vi "Lab1_task4.vi"() -> ()   [LabVIEW 2022 SP3]
uses:
  <vilib>/Utility/file.llb/Write Delimited Spreadsheet (DBL).vi
panel:
  in  "file path (dialog if empty)":path
  out "Waveform Graph":dbl[](graph)
  in  "Sampling Period (ms)":u32
  in  "Number of Samples":i32
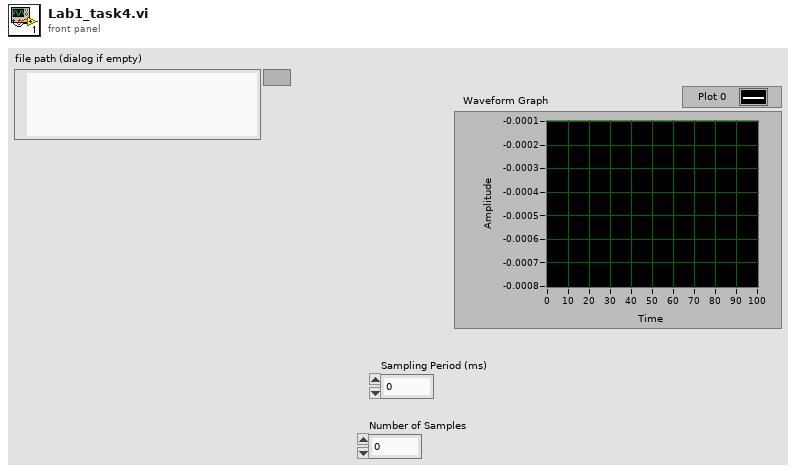
[diagram p1: front panel]
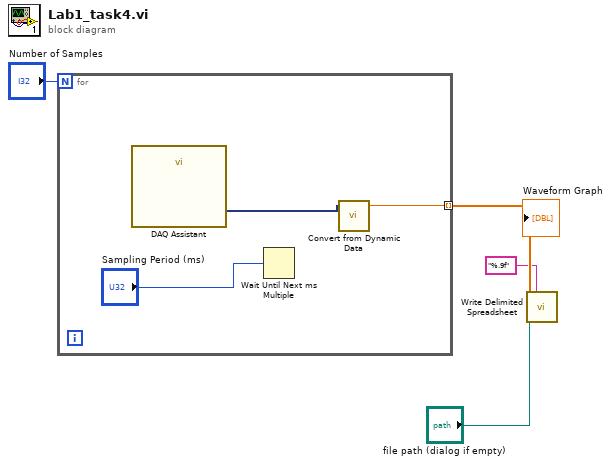
[diagram p0: block diagram]
diagram:
  n1 = for {
    N: "Number of Samples" -> [_]
    tunnel: [w5] -> w3 mode=indexing
    n2 = call "DAQ Assistant"() -> ("data"=w6:dynamicdata)  [unwired: 17 in, 2 out]
    n3 = Wait Until Next ms Multiple(millisecond multiple="Sampling Period (ms)") -> ()  [unwired: 1 out]
    n4 = call "Convert from Dynamic Data"("Dynamic Data Type"=w6) -> ("Scalar"=w5:dbl)  [unwired: 3 in]
  }
  "Waveform Graph" <- w3
  n5 = call-poly <vilib>:"Write Delimited Spreadsheet.vi"("file path (dialog if empty)"="file path (dialog if empty)", "format (%.3f)"="%.9f", "1D data"=w3) -> ()  [unwired: 11 in, 2 out]
